vi "Build String.vi"(7 "Section":string[](array[string]), 8 "error in (no error)":errorcluster, 9 "Content":T1[](array[typedef]), 10 "Keys":string[](array[string]), 11 "ConfigManager.Text in":refnum<class "ConfigManager.Text.lvclass">) -> (0 "error out":errorcluster, 2 "Input String":string, 3 "ConfigManager.Text out":refnum<class "ConfigManager.Text.lvclass">)   [LabVIEW 2013, in "CfgManager.Text.lvlib" / "ConfigManager.Text.lvclass"]
uses:
  ConfigManager.Text.lvclass
  Dictionary Payload -- cluster.ctl
  ConfigManager.Text.lvclass/ConfigManager.Text.ctl
  <vilib>/LabVIEW Open Source Project/Unicity/Delimiter/Delimiter.lvclass
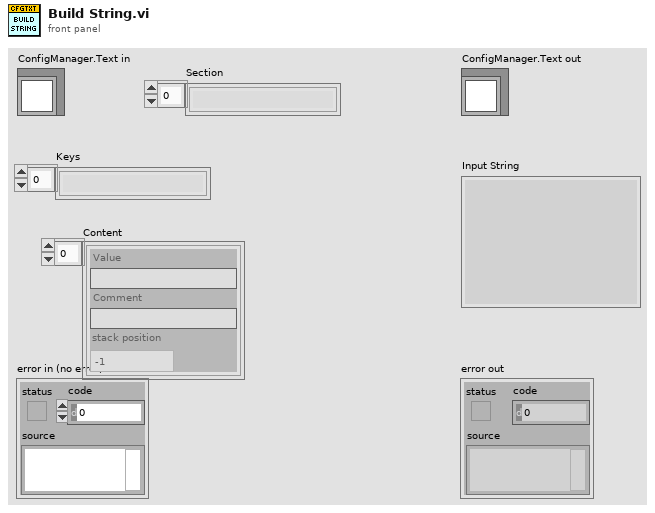
[diagram p1: front panel]
types:
  T1 = typedef "CfgManager.Text.lvlib/ConfigManager.Text.lvclass/Dictionary Payload -- cluster.ctl" = cluster{"Value":string, "Comment":string, "stack position":i32}
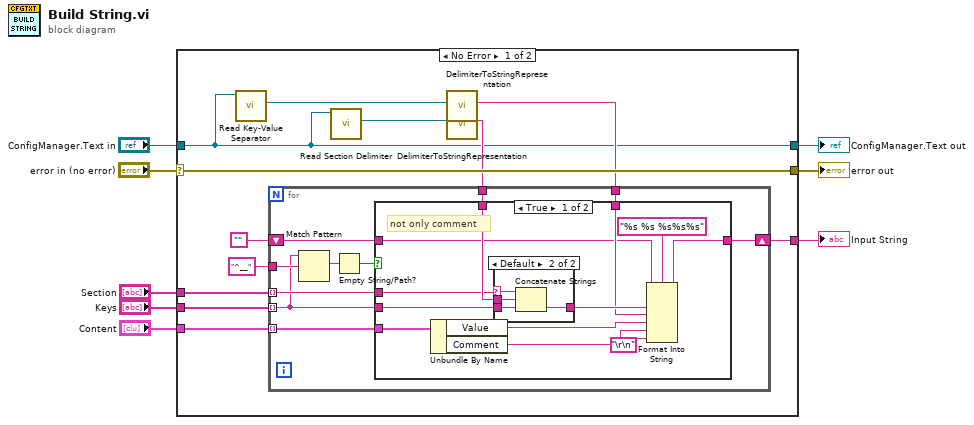
[diagram p0: block diagram]
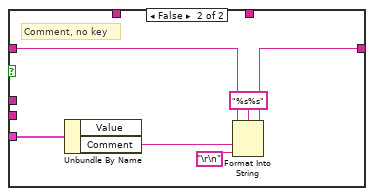
[diagram p3: hidden frame]
diagram:
  n1 = case shown="No Error" "error in (no error)" {
    selector: "error in (no error)" -> [w20 w55]
    tunnel: [w20 w55] -> w7
    tunnel: [w12 w54] -> w5
    tunnel: "ConfigManager.Text in" -> [w12 w54]
    tunnel: "Section" -> [w18 _]
    tunnel: "Keys" -> [w17 _]
    tunnel: "Content" -> [w16 _]
    tunnel: [w13 _] -> w1
    frame No Error {
      n2 = call "Read Key-Value Separator.vi"("ConfigManager.Text in"=w12) -> ("Key Value Separator"=w11:refnum<class "Delimiter.lvclass">)  [unwired: 9 in, 1 out]
      n3 = call "Read Section Delimiter.vi"("ConfigManager.Text in"=w12) -> ("Section Delimiter"=w10:refnum<class "Delimiter.lvclass">)  [unwired: 9 in, 1 out]
      n4 = call <vilib>:"DelimiterToStringRepresentation.vi"("Delimiter"=w11) -> ("String representation"=w14:string)  [unwired: 10 in]
      n5 = call <vilib>:"DelimiterToStringRepresentation.vi"("Delimiter"=w10) -> ("String representation"=w15:string)  [unwired: 10 in]
      n6 = for {
        shift-right: [w28] -> w13
        shift-left: "" -> [w26]
        tunnel: w18 -> [w23] mode=indexing
        tunnel: w17 -> [w21] mode=indexing
        tunnel: w16 -> [w27] mode=indexing
        tunnel: w15 -> [w30]
        tunnel: w14 -> [w29]
        tunnel: "^__" ("regular expression") -> [w25]
        n7 = Match Pattern(string=w21, regular expression=w25) -> (match substring=w24:string)  [unwired: 1 in, 3 out]
        n8 = Empty String/Path?(string/path=w24) -> (empty?=w22:bool)
        n9 = case shown="True" w22 {
          tunnel: w30 -> [w42 _]
          tunnel: w29 -> [w40 _]
          tunnel: [w39 w53] -> w28
          tunnel: w27 -> [w37 w51]
          tunnel: w26 -> [w33 w48]
          tunnel: w23 -> [w32 _]
          tunnel: w21 -> [w31 _]
          frame True {
            # "not only comment"
            n10 = Unbundle By Name(w37) -> ("Value"=w36:string, "Comment"=w35:string)
            n11 = case shown="Default" w32 {
              selector: w32 -> [_ w47]
              tunnel: w42 -> [_ w46]
              tunnel: w31 -> [w43 w45]
              tunnel: [w43 w44] -> w41
              frame "" {
              }
              frame Default {
                n12 = Concatenate Strings(w47, w46, w45) -> (w44:string)
              }
            }
            n13 = Format Into String(format string="%s %s %s%s%s", initial string=w33, w41, w40, w36, w35, "\r\n") -> (resulting string=w39:string)  [unwired: 1 in, 1 out]
          }
          frame False {
            # "Comment, no key"
            n14 = Unbundle By Name(w51) -> ("Comment"=w50:string)  [unwired: 1 out]
            n15 = Format Into String(format string="%s%s", initial string=w48, w50, "\r\n") -> (resulting string=w53:string)  [unwired: 1 in, 1 out]
          }
        }
      }
    }
    frame Error {
    }
  }
  "error out" <- w7
  "ConfigManager.Text out" <- w5
  "Input String" <- w1
